vi "Runtime_Close.vi"(8 "error in (no error)":errorcluster={"status"=FALSE, "code"=0, "source"="\"\""}, 10 "service references":string, 11 "Run state":string) -> (0 "error out":errorcluster={"status"=FALSE, "code"=0, "source"="\"\""}, 2 "status ok":bool, 3 "Close results":string)   [LabVIEW 2026]
doc: "INTENT: Orderly release of application services. LOGIC: After safe state stop executor, bridge worker, logging and transport; report residual faults."
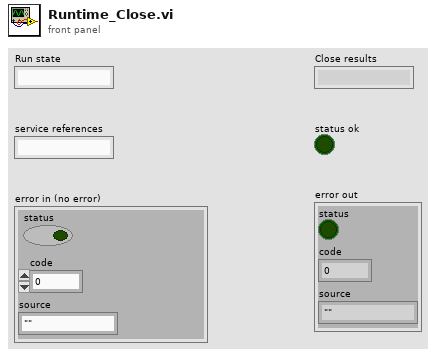
[diagram p1: front panel]
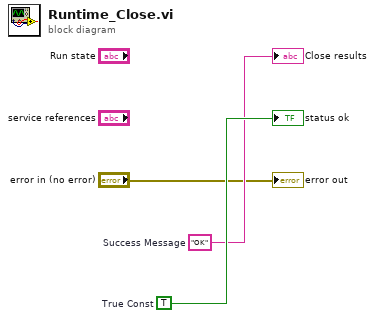
[diagram p0: block diagram]
diagram:
  w3 = TRUE  # True Const
  w2 = "OK"  # Success Message
  "Close results" <- w2
  "status ok" <- w3
  "error out" <- "error in (no error)"
